vi "NEO Swerve Drive.vi"(7 "Max V":dbl, 9 "Drive Conditions":T3, 10 "Robot Velocities":T8, 11 "Motors In":T4 {"Steer Scaling" format="%.2f"; "Drive Scaling" format="%.2f"; "Pod Locations (ft)"."Right Back" format="%.2f"; "Pod Locations (ft)"."Right Front" format="%.2f"; "Pod Locations (ft)"."Left Back" format="%.2f"; "Pod Locations (ft)"."Left Front" format="%.2f"}) -> (0 "Arbitrary":T1, 3 "Pod Setpoints (ft/s and deg)":T7)   [LabVIEW 2023]
uses:
  Type Definitions/Data/Pod Setpoints.ctl
  Type Definitions/Data/Pod Positions.ctl
  Type Definitions/Hardware/Swerve Drives/(NEO-NEO-ThroughBore-Pigeon2) Swerve.ctl
  Type Definitions/Data/Robot Velocities.ctl
  Drive Conditions.ctl
  <vilib>/REV Custom Controls/REVSparkRefnum.ctl
  <vilib>/REVLibDriver/REVLibDriver.lvlib
panel:
  out "Waveform Chart":T2(graph)
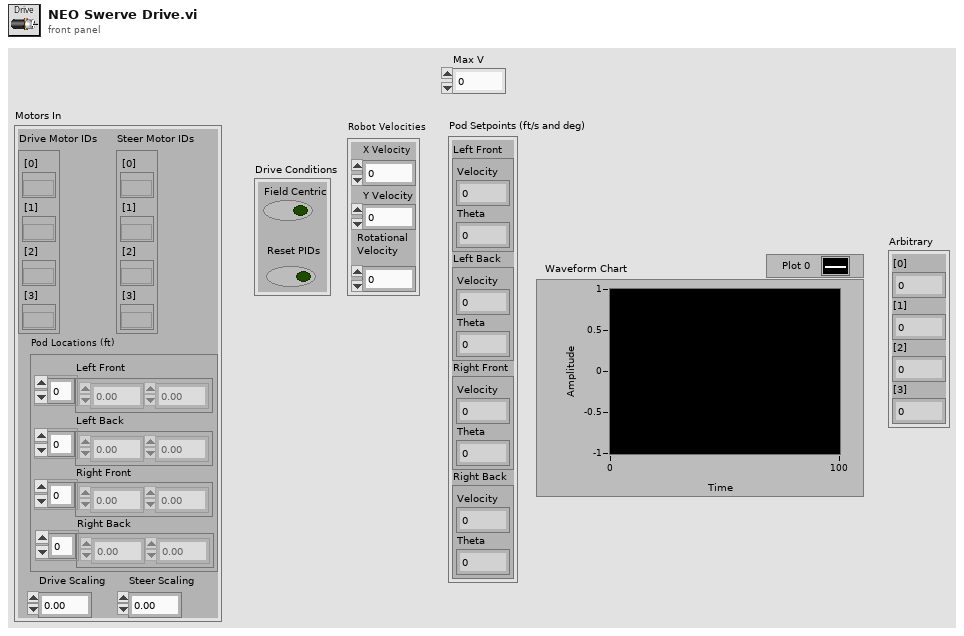
[diagram p1: front panel]
types:
  T1 = cluster{"[0]":dbl, "[1]":dbl, "[2]":dbl, "[3]":dbl}
  T2 = cluster{"Left Front":dbl, "Left Back":dbl, "Right Front":dbl, "Right Back":dbl}
  T3 = typedef "Drive Conditions.ctl" = cluster{"Field Centric":bool, "Reset PIDs":bool}
  T4 = typedef "(NEO-NEO-ThroughBore-Pigeon2) Swerve.ctl" = cluster{"Drive Motor IDs":cluster{"[0]":T5, "[1]":T5, "[2]":T5, "[3]":T5}, "Steer Motor IDs":cluster{"[0]":T5, "[1]":T5, "[2]":T5, "[3]":T5}, "Pod Locations (ft)":T6, "Drive Scaling":dbl, "Steer Scaling":dbl}
  T5 = typedef "REVLibDriver.lvlib/REVSparkRefnum.ctl" = refnum<k20>
  T6 = typedef "Pod Positions.ctl" = cluster{"Left Front":dbl[], "Left Back":dbl[], "Right Front":dbl[], "Right Back":dbl[]}
  T7 = typedef "Pod Setpoints.ctl" = cluster{"Left Front":cluster{"Velocity":dbl, "Theta":dbl}, "Left Back":cluster{"Velocity":dbl, "Theta":dbl}, "Right Front":cluster{"Velocity":dbl, "Theta":dbl}, "Right Back":cluster{"Velocity":dbl, "Theta":dbl}}
  T8 = typedef "Robot Velocities.ctl" = cluster{"X Velocity":dbl, "Y Velocity":dbl, "Rotational \nVelocity":dbl}
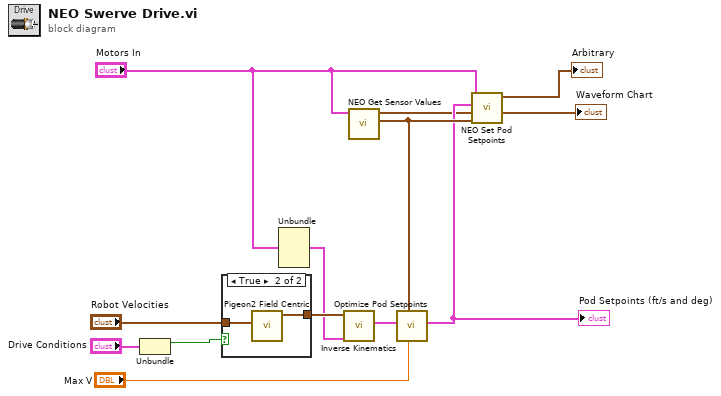
[diagram p0: block diagram]
diagram:
  n1 = Unbundle("Drive Conditions") -> ("Field Centric"=w7:bool)  [unwired: 1 out]
  n2 = case shown="True" w7 {
    tunnel: "Robot Velocities" -> [w13 w15]
    tunnel: [w13 w14] -> w4
    frame False {
    }
    frame True {
      n3 = call "Pigeon2 Field Centric.vi"("Field Centric Velocities"=w15) -> ("Robot Centric Velocities"=w14:T8)  [unwired: 10 in]
    }
  }
  n4 = Unbundle("Motors In") -> ("Pod Locations (ft)"=w3:T6)  [unwired: 4 out]
  n5 = call "Inverse Kinematics.vi"("Radii (ft)"=w3, "Target Velocity (ft/s and deg/s)"=w4) -> ("Pod Setpoints (ft/s and deg)"=w10:T7)  [unwired: 7 in, 2 out]
  n6 = call "NEO Get Sensor Values.vi"("Motors In"="Motors In") -> ("Steer Angles (degrees)"=w11:T2, "Drive Velocities (ft/s)"=w6:T2)  [unwired: 9 in]
  "Waveform Chart" <- w6
  n7 = call "Optimize Pod Setpoints.vi"("Max V"="Max V", "Current Pod Steering (deg)"=w11, "Initial Pod Setpoints (ft/s and deg)"=w10) -> ("Optimized Pod Setpoints (ft/s and deg)"=w9:T7)  [unwired: 8 in]
  "Pod Setpoints (ft/s and deg)" <- w9
  n8 = call "NEO Set Pod Setpoints.vi"("Steer Angles (degrees)"=w11, "Drive Velocities (ft/s)"=w6, "Pod Setpoints (ft/s and deg)"=w9, "Motors In"="Motors In") -> ("Arbitrary"=→"Arbitrary":T1)  [unwired: 7 in]
